vi "Groups.vi"(8 "error in (no error)":errorcluster, 11 "Task in":refnum<class "Task Config.lvclass">) -> (0 "error out":errorcluster, 2 "Groups":refnum<class "Group Config.lvclass">[](array[class]), 3 "Task out":refnum<class "Task Config.lvclass">)   [LabVIEW 2020, in "VolatusConfig.lvlib" / "Task Config.lvclass"]
uses:
  Task Config.lvclass
  C:/dev/lv20CE/relink/lv-volatus/VolatusConfig/VolatusConfigElement/VolatusConfigElement.lvclass
  Group/Group Config.lvclass
  Meta Type.ctl
  VolatusConfigElement/VolatusConfigElement.lvclass/VolatusConfigElement.ctl
  VolatusConfigElement/Element.vi
  lv-cdm/CDM-Config/Config Lookup/Match Meta.vi
  lv-cdm/CDM-Config/Config Element/Owner.vi
  lv-cdm/CDM-Config/Config Manager/Lookup Descendant.vi
  lv-cdm/CDM-Config/Config Filter/Config Lookup.lvclass
  Task Config.lvclass/Task Config.ctl
  VolatusConfig.lvlib
  VolatusConfigElement/VolatusConfigElement.lvclass
  C:/dev/lv20CE/relink/lv-volatus/VolatusConfig/Task/Task Config.lvclass
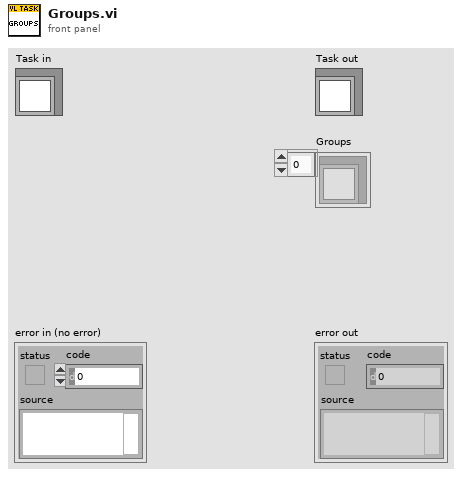
[diagram p1: front panel]
types:
  T1 = typedef "VolatusConfig.lvlib/Meta Type.ctl" = enum16{"UNKNOWN", "VL_System", "VL_Cluster", "VL_Node", "VL_Task", "VL_Group", "VL_Channel", "VL_Task_List", "VL_Scaling", "VL_Sensor", "VL_Sensor_List", "VL_Scale"}
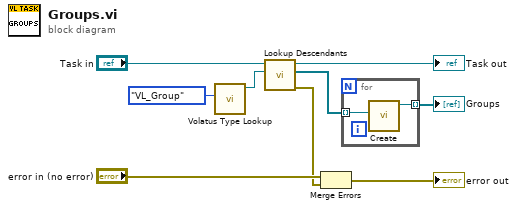
[diagram p0: block diagram]
diagram:
  n1 = call "Volatus Type Lookup.vi"("Meta Type"=Meta_Type."VL_Group") -> ("Config Lookup out"=w3:refnum<class "Config Lookup.lvclass">)  [unwired: 9 in, 1 out]
  n2 = call "Lookup Descendants.vi"("Lookup"=w3, "VolatusConfigElement in"="Task in") -> ("error out"=w2:errorcluster, "Descendants"=w1:refnum<class "Config Element.lvclass">[], "VolatusConfigElement out"=→"Task out":refnum<class "Task Config.lvclass">)  [unwired: 7 in]
  n3 = Merge Errors("error in (no error)", w2) -> (→"error out":errorcluster)
  n4 = for {
    tunnel: w1 -> [w11] mode=indexing
    tunnel: [w10] -> w6 mode=indexing
    n5 = call "Create.vi"("Element"=w11) -> ("Group out"=w10:refnum<class "Group Config.lvclass">)  [unwired: 9 in, 1 out]
  }
  "Groups" <- w6
